vi "Save Object as VI.vi"(8 "error in (no error)":errorcluster, 9 "Name":string, 11 "Object in":refnum<vi>) -> (0 "error out":errorcluster, 3 "Object out":refnum<vi>, 5 "Ok?":bool)   [LabVIEW 2020]
uses:
  <vilib>/Utility/miscctls.llb/LVPositionTypeDef.ctl
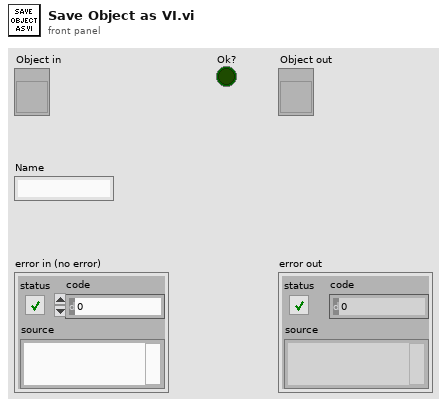
[diagram p1: front panel]
types:
  T1 = typedef "LVPositionTypeDef.ctl" = cluster{"Left":i32, "Top":i32}
  T2 = typedef "imagedata.ctl" = cluster{"image type":i32, "image depth":i32, "image":u8[], "mask":u8[], "colors":u32[], "Rectangle":cluster{"left":i16, "top":i16, "right":i16, "bottom":i16}}
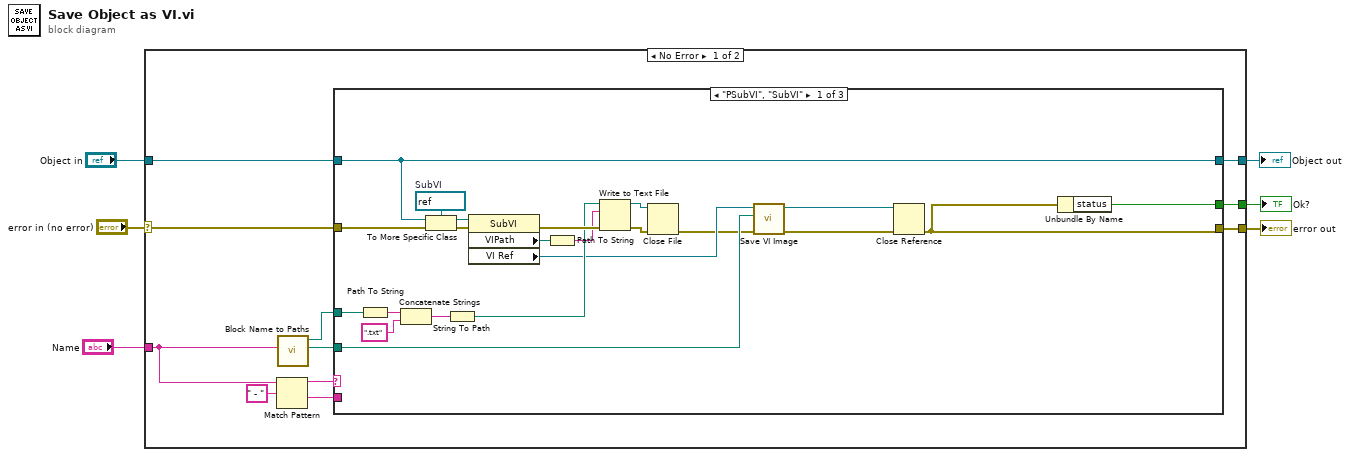
[diagram p0: block diagram]
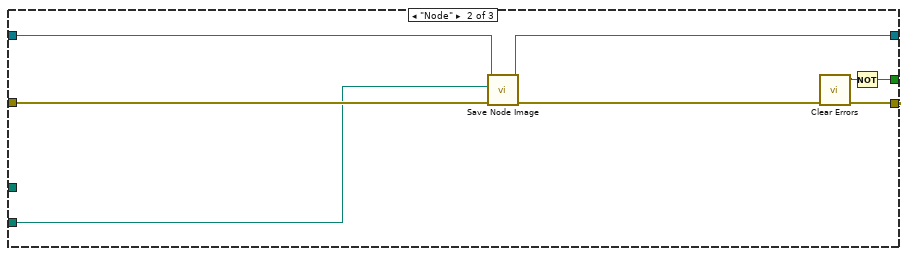
[diagram p2: hidden frame]
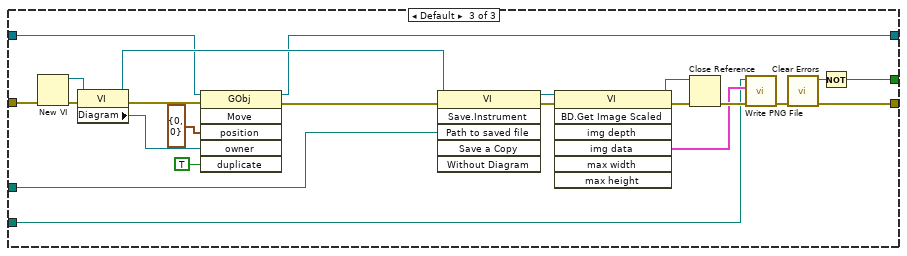
[diagram p3: hidden frame]
diagram:
  n1 = case shown="No Error" "error in (no error)" {
    selector: "error in (no error)" -> [w17 w73]
    tunnel: [w16 w73] -> w6
    tunnel: [w15 FALSE ("specific error cleared?")] -> w4
    tunnel: [w10 w71] -> w3
    tunnel: "Object in" -> [w9 w71]
    tunnel: "Name" -> [w7 _]
    frame No Error {
      n2 = Match Pattern(string=w7, regular expression=" - ") -> (before substring=w13:string, after substring=w8:string)  [unwired: 1 in, 2 out]
      n3 = call "Block Name to Paths.vi"("Block Name"=w7) -> ("Image Path"=w11:path, "Block Path"=w12:path)  [unwired: 9 in]
      n4 = case shown="\"PSubVI\", \"SubVI\"" w13 {
        tunnel: w17 -> [w36 w44 w56]
        tunnel: [w23 w46 w54] -> w16
        tunnel: [w24 w45 w52] -> w15
        tunnel: w12 -> [w35 _ w51]
        tunnel: w11 -> [w22 w40 w50]
        tunnel: w9 -> [w25 w42 w49]
        tunnel: [w25 w41 w48] -> w10
        tunnel: w8 -> [_ _ _]
        frame "PSubVI", "SubVI" {
          w39 = refnum<vi> refnum  # SubVI
          n5 = Path To String(path=w35) -> (string=w34:string)
          n6 = Concatenate Strings(w34, ".txt" ("string")) -> (w31:string)
          n7 = To More Specific Class(target class=w39, reference=w25, error in=w36) -> (specific class reference=w37:refnum<vi>, error out=w38:errorcluster)
          n8 = String To Path(string=w31) -> (path=w30:path)
          n9 = property on="Property Node" class="SubVI"(reference=w37, error in=w38) -> (error out=w32:errorcluster, "VIPath"=w29:path, "VI Ref"=w21:refnum<vi>)  [unwired: 1 out]
          n10 = Path To String(path=w29) -> (string=w28:string)
          n11 = Write to Text File(file (use dialog)=w30, text=w28, error in=w32) -> (refnum out=w26:refnum<file>, error out=w27:errorcluster)  [unwired: 1 in, 1 out]
          n12 = Close File(refnum=w26, error in=w27) -> (error out=w19:errorcluster)  [unwired: 1 out]
          n13 = call "Save VI Image.vi"("error in (no error)"=w19, "Image Path"=w22, "VI in"=w21) -> ("error out"=w18:errorcluster, "VI out"=w20:refnum<vi>)  [unwired: 7 in]
          n14 = Close Reference(reference=w20, error in (no error)=w18) -> (error out=w23:errorcluster)
          n15 = Unbundle By Name(w23) -> ("status"=w24:bool)
        }
        frame "Node" {
          n16 = call "Save Node Image.vi"("error in (no error)"=w44, "Image Path"=w40, "Object in"=w42) -> ("error out"=w43:errorcluster, "Object out"=w41:refnum<vi>)  [unwired: 7 in]
          n17 = call <vilib>:"Clear Errors.vi"("error in (no error)"=w43) -> ("error out"=w46:errorcluster, "specific error cleared?"=w47:bool)  [unwired: 5 in]
          n18 = Not(x=w47) -> (.not. x?=w45:bool)
        }
        frame Default {
          n19 = New VI(8:w56) -> (0:w69:errorcluster, 3:w70:refnum<vi>)  [unwired: 6 in]
          n20 = property class="VI"(reference=w70, error in=w69) -> (reference out=w65:refnum<vi>, error out=w59:errorcluster, "Diagram"=w66:refnum<vi>)
          n21 = invoke class="GObj" method="Move"(reference=w49, error in=w59, "position"=T1 {"Left"=0, "Top"=0}, "owner"=w66, "duplicate"=TRUE ("Duplicate? (F)")) -> (reference out=w48:refnum<vi>, error out=w64:errorcluster)  [unwired: 1 in, 4 out]
          n22 = invoke class="VI" method="Save.Instrument"(reference=w65, error in=w64, "Path to saved file"=w51) -> (reference out=w63:refnum<vi>, error out=w61:errorcluster)  [unwired: 3 in, 4 out]
          n23 = invoke class="VI" method="BD.Get Image Scaled"(reference=w63, error in=w61) -> (reference out=w62:refnum<vi>, error out=w60:errorcluster, "img data"=w57:T2)  [unwired: 5 in, 4 out]
          n24 = Close Reference(reference=w62, error in (no error)=w60) -> (error out=w58:errorcluster)
          n25 = call <vilib>:"Write PNG File.vi"("error in (no error)"=w58, "image data"=w57, "path to PNG file"=w50) -> ("error out"=w55:errorcluster)  [unwired: 7 in, 1 out]
          n26 = call <vilib>:"Clear Errors.vi"("error in (no error)"=w55) -> ("error out"=w54:errorcluster, "specific error cleared?"=w53:bool)  [unwired: 5 in]
          n27 = Not(x=w53) -> (.not. x?=w52:bool)
        }
      }
    }
    frame Error {
    }
  }
  "error out" <- w6
  "Ok?" <- w4
  "Object out" <- w3
